vi "Liste mails.vi"() -> ()   [LabVIEW 2022 SP3]
uses:
  Enum/Enum 11.ctl
  Variables globales/Variable glob mails.vi
  <vilib>/Utility/config.llb/Write Key (String).vi
  <vilib>/Utility/config.llb/NI_LVConfig.lvlib
panel:
  out "référence au VI":refnum<vi>
  in  "annuler":bool
  in  "sortir":bool
  in  "Autres adresses mail":string[](array[string])
  in  "Adresses mail liste :":i32[](listbox)=[5]
  # "Sélection des mails\npour envoi\nalertes régulateurs et surveillances"
  # "Ce logiciel et les informations qu'il contient, sont la propriété de l’IAS et ne peuvent être diffusés sans l’autorisation de la Station d’étalonnage"
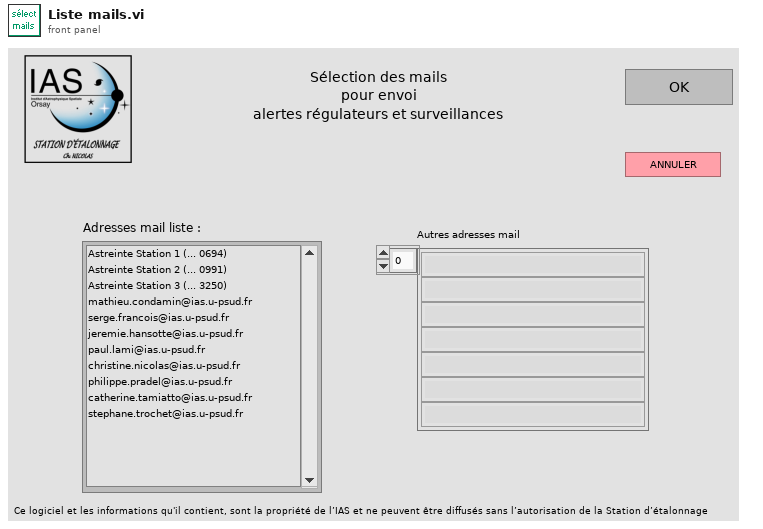
[diagram p1: front panel]
types:
  T1 = typedef "Enum 11.ctl" = enum16{"init", "mails", "choix", "enregistrer", "fin"}
  T2 = enum32{"Invalid", "Standard", "Closed", "Hidden", "Minimized", "Maximized"}
  T3 = typedef "NI_LVConfig.lvlib/Config Data RefNum.ctl" = refnum<k1>
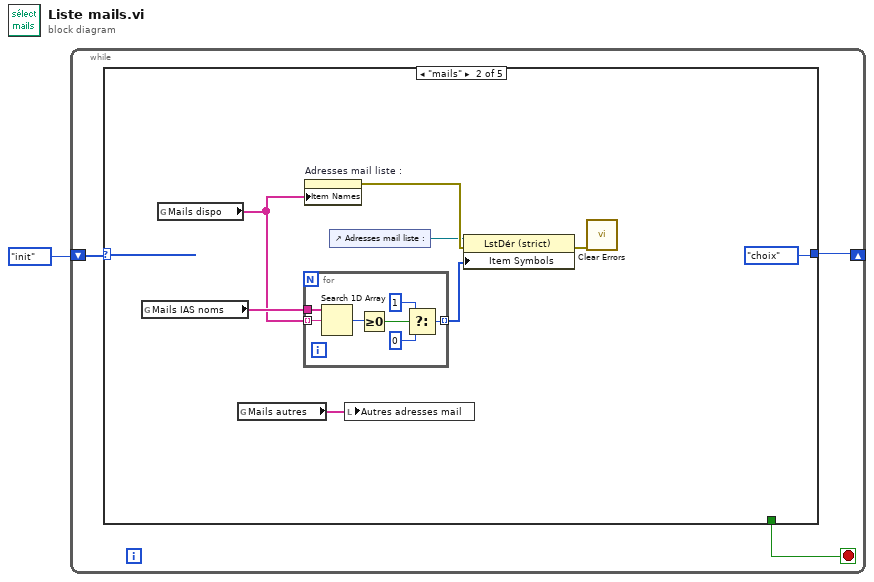
[diagram p0: block diagram]
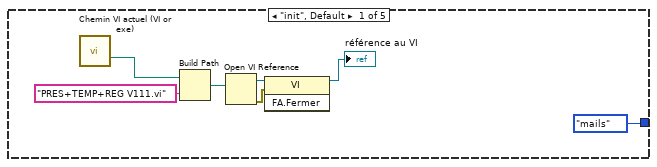
[diagram p2: hidden frame]
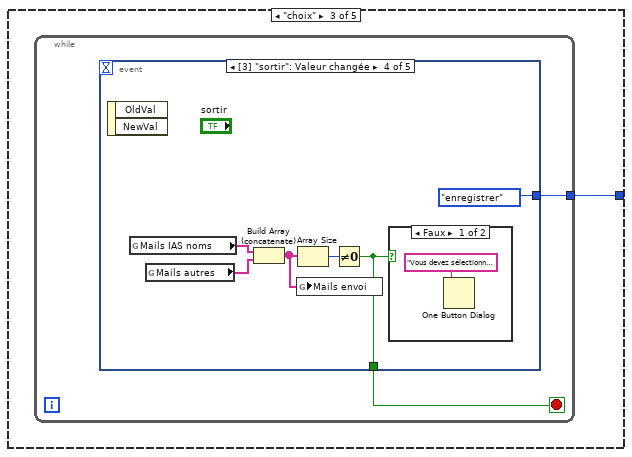
[diagram p3: hidden frame]
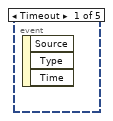
[diagram p4: hidden frame]
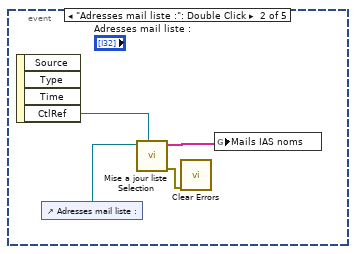
[diagram p5: hidden frame]
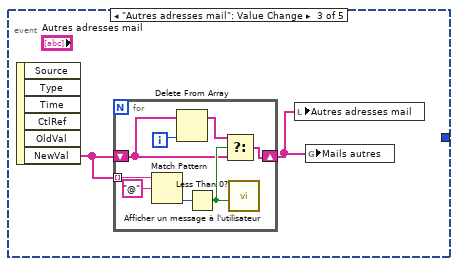
[diagram p6: hidden frame]
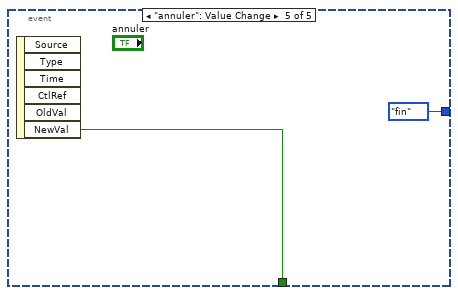
[diagram p8: hidden frame]
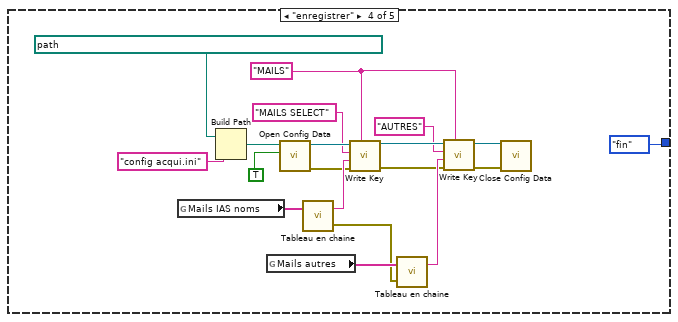
[diagram p9: hidden frame]
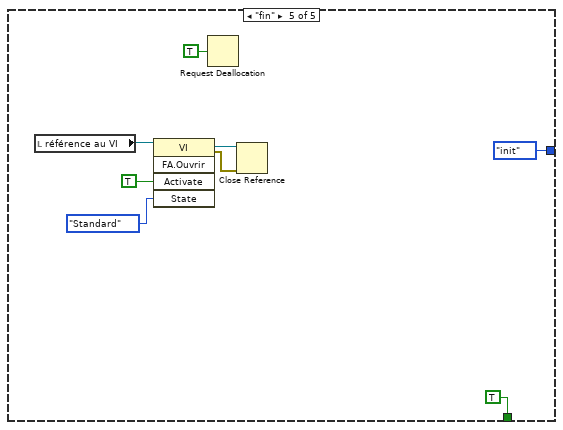
[diagram p10: hidden frame]
diagram:
  n1 = while {
    shift-right: [w3] -> _
    shift-left: Enum_11."init" ("Énum") -> [w4]
    stop <- w2 stop-if-true
    n2 = case shown="\"mails\"" w4 {
      tunnel: [Enum_11."mails" ("Énum") Enum_11."choix" ("Énum") w27 Enum_11."fin" ("Énum") Enum_11."init" ("Énum")] -> w3
      tunnel: [_ _ _ _ TRUE] -> w2
      frame "init", Default {
        n3 = call "Chemin VI actuel (VI or exe).vi"() -> ("VI or executable installation directory"=w10:path)  [unwired: 14 in, 1 out]
        n4 = Build Path(base path=w10, name or relative path="PRES+TEMP+REG V111.vi" ("nom ou chemin relatif")) -> (appended path=w7:path)
        n5 = Open VI Reference(vi path=w7) -> (vi reference=w6:refnum<vi>, error out=w5:errorcluster)  [unwired: 5 in]
        n6 = invoke class="VI" method="FA.Fermer"(reference=w6, error in=w5) -> (reference out=→"référence au VI":refnum<vi>)  [unwired: 1 in, 2 out]
      }
      frame "mails" {
        n7 = global read "Variable glob mails.vi" "Mails IAS noms"() -> (w14:string[])
        n8 = global read "Variable glob mails.vi" "Mails dispo"() -> (w12:string[])
        n9 = global read "Variable glob mails.vi" "Mails autres"() -> (w13:string[])
        n10 = for {
          tunnel: w14 -> [w26]
          tunnel: w12 -> [w25] mode=indexing
          tunnel: [w20] -> w17 mode=indexing
          n11 = Search 1D Array(1D array=w26, element=w25) -> (index of element=w24:i32)  [unwired: 1 in]
          n12 = Greater Or Equal To 0?(x=w24) -> (x >= 0?=w23:bool)
          n13 = Select(t=1 ("cas vrai"), s=w23, f=0) -> (s? t:f=w20:i32)
        }
        n14 = property on="Adresses mail liste :" class="LstDér (strict)"("Item Names"=w12) -> (error out=w18:errorcluster)  [unwired: 2 in, 1 out]
        n15 = control-ref of="Adresses mail liste :"() -> (w16:refnum<vi>)
        n16 = local write "Autres adresses mail"(w13) -> ()
        n17 = property class="LstDér (strict)"(reference=w16, error in=w18, "Item Symbols"=w17) -> (error out=w19:errorcluster)  [unwired: 1 out]
        n18 = call <vilib>:"Clear Errors.vi"("error in (no error)"=w19) -> ()  [unwired: 5 in, 2 out]
      }
      frame "choix" {
        n19 = while {
          tunnel: [w28] -> w27
          stop <- w29 stop-if-true
          n20 = event shown="[3] \"sortir\": Valeur changée" {
            selector: _ -> [_ _ _ _ _]
            dyn-events: _ -> [_ _ _ _ _]
            timeout: _ -> [_ _ _ _ _]
            tunnel: [_ _ _ w48 w52] -> w29
            tunnel: [_ _ _ Enum_11."enregistrer" ("Énum") Enum_11."fin" ("Énum")] -> w28
            event Timeout {
              n21 = event-data() -> ()  [unwired: 1 in, 3 out]
            }
            event "Adresses mail liste :": Double Click {
              n22 = event-data() -> ("CtlRef"=w32:refnum<vi>)  [unwired: 1 in, 3 out]
              n23 = control-ref of="Adresses mail liste :"() -> (w31:refnum<vi>)
              n24 = call "Mise a jour liste Selection.vi"("RéfCmde sélection"=w32, "Choisir capteur parmis"=w31) -> ("error out"=w33:errorcluster, "Capteurs choisit"=w30:string[])  [unwired: 8 in]
              n25 = call <vilib>:"Clear Errors.vi"("error in (no error)"=w33) -> ()  [unwired: 5 in, 2 out]
              n26 = global write "Variable glob mails.vi" "Mails IAS noms"(w30) -> ()
            }
            event "Autres adresses mail": Value Change {
              n27 = event-data() -> ("NewVal"=w35:string[])  [unwired: 1 in, 5 out]
              n28 = for {
                tunnel: w35 -> [w43] mode=indexing
                shift-right: [w39] -> w34
                shift-left: w35 -> [w38]
                i -> [w37]
                n29 = Match Pattern(string=w43, regular expression="@" ("expression régulière")) -> (offset past match=w41:i32)  [unwired: 1 in, 3 out]
                n30 = Delete From Array(array=w38, index=w37) -> (array with subset deleted=w36:string[])  [unwired: 1 in, 1 out]
                n31 = Less Than 0?(x=w41) -> (x < 0?=w40:bool)
                n32 = Select(t=w36, s=w40, f=w38) -> (s? t:f=w39:string[])
                n33 = call "Afficher un message à l'utilisateur"("Enable"=w40) -> ()  [unwired: 9 in, 2 out]
              }
              n34 = local write "Autres adresses mail"(w34) -> ()
              n35 = global write "Variable glob mails.vi" "Mails autres"(w34) -> ()
            }
            event "sortir": Value Change {
              n36 = event-data() -> ()  [unwired: 1 in, 2 out]
              n37 = global read "Variable glob mails.vi" "Mails IAS noms"() -> (w44:string[])
              n38 = global read "Variable glob mails.vi" "Mails autres"() -> (w45:string[])
              n39 = Build Array (concatenate)(w44, w45) -> (w46:string[])
              n40 = global write "Variable glob mails.vi" "Mails envoi"(w46) -> ()
              n41 = Array Size(array=w46) -> (size(s)=w49:i32)
              n42 = Not Equal To 0?(x=w49) -> (x != 0?=w48:bool)
              n43 = case shown="Faux" w48 {
                frame False {
                  n44 = One Button Dialog(message="Vous devez sélectionner au moins une adresse mail") -> ()  [unwired: 1 in, 1 out]
                }
                frame True {
                }
              }
            }
            event "annuler": Value Change {
              n45 = event-data() -> ("NewVal"=w52:bool)  [unwired: 1 in, 5 out]
            }
          }
        }
      }
      frame "enregistrer" {
        w68 = "MAILS" ("section")
        n46 = global read "Variable glob mails.vi" "Mails IAS noms"() -> (w55:string[])
        n47 = Build Path(base path=path "C:/LABVIEW/PRES+TEMP+REG dernière version/Configurations", name or relative path="config acqui.ini" ("nom ou chemin relatif")) -> (appended path=w61:path)
        n48 = global read "Variable glob mails.vi" "Mails autres"() -> (w54:string[])
        n49 = call <vilib>:"Open Config Data.vi"("create file if necessary (T)"=TRUE ("create file if necessary? (T)"), "configuration file path"=w61) -> ("error out"=w65:errorcluster, "refnum"=w64:T3)  [unwired: 7 in, 1 out]
        n50 = call "Tableau en chaine.vi"("Tableau 1D"=w55) -> ("error out"=w53:errorcluster, "Chaîne"=w70:string)  [unwired: 1 in]
        n51 = call-poly <vilib>:"Write Key.vi"("section"=w68, "error in (no error)"=w65, "value"=w70, "key"="MAILS SELECT", "refnum"=w64) -> ("error out"=w67:errorcluster, "refnum out"=w66:T3)  [unwired: 4 in, 1 out]
        n52 = call "Tableau en chaine.vi"("error in (no error)"=w53, "Tableau 1D"=w54) -> ("Chaîne"=w71:string)  [unwired: 1 out]
        n53 = call-poly <vilib>:"Write Key.vi"("section"=w68, "error in (no error)"=w67, "value"=w71, "key"="AUTRES", "refnum"=w66) -> ("error out"=w58:errorcluster, "refnum out"=w57:T3)  [unwired: 4 in, 1 out]
        n54 = call <vilib>:"Close Config Data.vi"("error in (no error)"=w58, "refnum"=w57) -> ()  [unwired: 8 in, 2 out]
      }
      frame "fin" {
        n55 = local read "référence au VI"() -> (w74:refnum<vi>)
        n56 = invoke class="VI" method="FA.Ouvrir"(reference=w74, "Activate"=TRUE ("Activer ?"), "State"=T2."Standard" ("État")) -> (reference out=w76:refnum<vi>, error out=w75:errorcluster)  [unwired: 2 in, 3 out]
        n57 = Request Deallocation(TRUE ("flag")) -> ()
        n58 = Close Reference(reference=w76, error in (no error)=w75) -> ()  [unwired: 1 out]
      }
    }
  }
